vi "Read Configuration File.vi"(8 "error in (no error)":errorcluster, 11 "Instrument.Lockin":refnum<class "Instrument.Lockin.lvclass">) -> (0 "error out":errorcluster, 3 "Instrument.Lockin out":refnum<class "Instrument.Lockin.lvclass">)   [LabVIEW 2019, in "Instrument.Lockin.lvlib" / "Instrument.Lockin.lvclass"]
uses:
  Instrument.Lockin.lvclass
  C:/Program Files (x86)/National Instruments/LabVIEW 2019/user.lib/LevyLab/Instrument Framework/Instrument/Instrument.lvclass
  <userlib>/LevyLab/Instrument Framework/Instrument/Instrument.lvclass/Instrument.ctl
  <userlib>/LevyLab/Configuration/Configuration.lvclass/Configuration.ctl
  Instrument.Lockin.lvclass/Instrument.Lockin.ctl
  <userlib>/LevyLab/Configuration/Write Section.vi
  <userlib>/LevyLab/Instrument Framework/Instrument/Instrument.lvclass
  C:/Program Files (x86)/National Instruments/LabVIEW 2019/vi.lib/JKI/JKI SMO/SMO/SMO.lvclass
  <vilib>/JKI/JKI SMO/SMO/Protected/ThisLevelClassName.vi
  <userlib>/LevyLab/Instrument Framework/Instrument Types/Lockin/Instrument.LockinAPI.lvclass
  <userlib>/LevyLab/Configuration/Configuration.lvclass
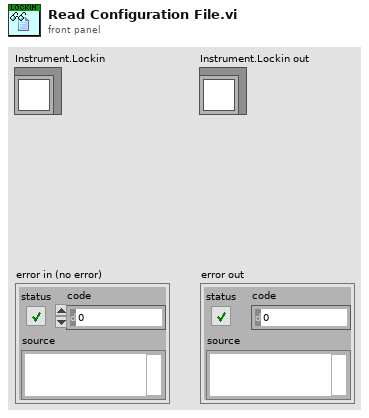
[diagram p1: front panel]
types:
  T1 = typedef "Instrument.Lockin.lvlib/Instrument.Lockin.lvclass/Lockin.Logging Mode--Enum.ctl" = enum16{"enabled", "disabled"}
  T2 = typedef "Instrument.Lockin.lvlib/Instrument.Lockin.lvclass/Lockin.LogPaths.Data--Cluster.ctl" = cluster{"PXI":cluster{"System Serial Number (text)":string, "Channel (i32)":string, "Channel Type (text)":string, "Data (dbl)":string, "Sweeping? (bool)":string}, "MCLI":cluster{"System Serial Number (text)":string, "System Channel (i32)":string, "Ref Channel (i32)":string, "X Data (dbl)":string, "Y Data (dbl)":string, "Sweeping? (bool)":string}}
  T3 = typedef "Instrument.Lockin.lvlib/Instrument.Lockin.lvclass/Lockin.LogPaths.Configuration--Cluster.ctl" = cluster{"Systems":cluster{"System Serial Number (text)":string, "Chassis Serial Number (text)":string, "Chassis Type (text)":string, "Sample Rate (dbl)":string}, "Devices":cluster{"System Serial Number (text)":string, "Chassis Serial Number (text)":string, "Device Serial Number (text)":string, "Device Type (text)":string, "Chassis Slot (i32)":string, "Device Temperature (dbl)":string, "Device Calibration Temperature (dbl)":string, "Device Calibration Time (timestamptz)":string}, "Channels":cluster{"System Serial Number (text)":string, "System Channel (i32)":string, "Device Serial Number (text)":string, "Device Channel (i32)":string, "Channel Type (text)":string, "Channel Coupling (text)":string, "Channel Range (text)":string, "Channel Configuration (text)":string}, "MCLI":cluster{"System Serial Number (text)":string, "Software Version (text)":string, "REF Channel (i32)":string, "frequency (dbl)":string, "time constant (dbl)":string, "roll-off (i32)":string}}
  T4 = cluster{"Loggin mode":T1, "Logging interval (ms)":u32, "Data Log Paths":T2, "Config Log Paths":T3}
  T5 = typedef "Instrument.Lockin.lvlib/Instrument.DAQ.lvclass/Configuration--Cluster.ctl" = cluster{"DAQ":T6, "Channels":T21, "Prefilter":T29, "Offset and Gain":T30, "Amplitude Limit":T33, "DC Limit":T34, "Link Frequencies":T35, "Sweep":T36, "Duty Cycle":T40}
  T6 = typedef "Instrument.Lockin.lvlib/Instrument.DAQ.lvclass/Configuration.DAQ--Cluster.ctl" = cluster{"Sampling":T7, "Simulation mode":T10, "AI":T11, "AO":T16, "Calibration":T18, "Devices":T20[]}
  T7 = typedef "Instrument.Lockin.lvlib/Instrument.DAQ.lvclass/DAQ.Sampling--Cluster.ctl" = cluster{"Sampling":T8, "sample mode":i32, "Fs Mode":T9, "Fs Multiplier":dbl, "Refresh Rate (Hz)":dbl, "Decimation.PreDSP":i32, "Decimation.PostDSP":i32, "Fs.Output":dbl}
  T8 = typedef "Instrument.Lockin.lvlib/Instrument.DAQ.lvclass/DAQ.Sampling.Sampling--Cluster.ctl" = cluster{"Fs":dbl, "#s":i32}
  T9 = typedef "Instrument.Lockin.lvlib/Instrument.DAQ.lvclass/DAQ.Sampling.Fs Mode--enum.ctl" = enum16{"Manual", "Auto Fs", "Max Fs"}
  T10 = typedef "Instrument.Lockin.lvlib/Instrument.DAQ.lvclass/Simulation Mode--enum.ctl" = enum16{"AI = HW simulated", "AI = noise*AO", "AI = waveguide"}
  T11 = typedef "Instrument.Lockin.lvlib/Instrument.DAQ.lvclass/DAQ.Config.AI--Cluster--Array.ctl" = cluster{"Channels":tag, "Coupling":T12, "Range":T13, "terminal configuration":T14, "Type":T15}[]
  T12 = typedef "Instrument.Lockin.lvlib/Instrument.DAQ.lvclass/DAQ.Config.AI.Coupling--enum.ctl" = u16
  T13 = typedef "Instrument.Lockin.lvlib/Instrument.DAQ.lvclass/DAQ.Config.AI.Range--enum.ctl" = enum16{"±0.316", "±1.00", "±3.16", "±10.0", "±31.6", "±42.4", ""}
  T14 = typedef "Instrument.Lockin.lvlib/Instrument.DAQ.lvclass/DAQ.TerminalConfiguration--ring.ctl" = i32
  T15 = typedef "Instrument.Lockin.lvlib/Instrument.DAQ.lvclass/DAQ.Type--enum.ctl" = enum16{"None", "USB-4431", "PXI-446x"}
  T16 = typedef "Instrument.Lockin.lvlib/Instrument.DAQ.lvclass/DAQ.Config.AO--Cluster--Array.ctl" = cluster{"Channels":tag, "Range":T17, "terminal configuration":T14, "Type":T15}[]
  T17 = typedef "Instrument.Lockin.lvlib/Instrument.DAQ.lvclass/DAQ.Config.AO.Range--enum.ctl" = enum16{"±0.1", "±1.0", "±10.0", ""}
  T18 = typedef "Instrument.Lockin.lvlib/Instrument.DAQ.lvclass/DAQ.Calibration--Cluster--Array.ctl" = T19[]
  T19 = typedef "Instrument.Lockin.lvlib/Instrument.DAQ.lvclass/DAQ.Calibration--Cluster.ctl" = cluster{"Active Device":string, "SelfCal.LastDate/Time":dbl, "SelfCal.LastTemp":dbl, "DevTemp":dbl, "calibration due?":bool}
  T20 = typedef "Instrument.Lockin.lvlib/Instrument.DAQ.lvclass/DeviceInfo--Cluster.ctl" = cluster{"DeviceName":string, "DevIsSimulated":bool, "DeviceSerialNumber":string, "ProductType":string, "ProductCategory":i32, "ProductNumber":u32, "ChassisNumber":u32, "SlotNumber":u32, "ChassisName":string, "ChassisSerialNumber":string, "DevTemp":dbl, "SelfCal.LastDate/Time":string, "SelfCal.LastTemp":dbl, "calibration due?":bool}
  T21 = typedef "Instrument.Lockin.lvlib/Instrument.DAQ.lvclass/Configuration.Channels--Cluster.ctl" = cluster{"Cfg_AO":T22, "Cfg_AI":T25, "Cfg_REF":T27}
  T22 = typedef "Instrument.Lockin.lvlib/Instrument.DAQ.lvclass/AO.Channel--Cluster--Array.ctl" = T23[]
  T23 = typedef "Instrument.Lockin.lvlib/Instrument.DAQ.lvclass/AO.Channel--Cluster.ctl" = cluster{"Enable?":bool, "Channel":i32, "Amplitude":dbl, "Offset":dbl, "Frequency":dbl, "Phase":dbl, "Function":T24, "Sweeping?":bool, "Limit AC":bool, "Limit DC?":bool, "Duty Cycle":bool}
  T24 = typedef "Instrument.Lockin.lvlib/Instrument.DAQ.lvclass/AO.Channel.Function--Enum.ctl" = enum16{"sine", "square", "triangle", "saw"}
  T25 = typedef "Instrument.Lockin.lvlib/Instrument.DAQ.lvclass/AI.Channel--Cluster--Array.ctl" = T26[]
  T26 = typedef "Instrument.Lockin.lvlib/Instrument.DAQ.lvclass/AI.Channel--Cluster.ctl" = cluster{"Enable?":bool, "Channel":i32, "References":u16[], "reference index":i32}
  T27 = typedef "Instrument.Lockin.lvlib/Instrument.DAQ.lvclass/REF.Channel--Cluster--Array.ctl" = T28[]
  T28 = typedef "Instrument.Lockin.lvlib/Instrument.DAQ.lvclass/REF.Channel--Cluster.ctl" = cluster{"Enable?":bool, "Channel":i32, "Frequency":dbl, "Phase":dbl, "TC":dbl, "Roll-Off":i32}
  T29 = typedef "Instrument.Lockin.lvlib/Instrument.DAQ.lvclass/Configuration.Prefilter--Cluster.ctl" = cluster{"60 Hz":bool, "Low Pass":bool, "Low Pass Cutoff (Hz)":dbl}
  T30 = typedef "Instrument.Lockin.lvlib/Instrument.DAQ.lvclass/Channel.GainsAndOffsets--Cluster.ctl" = cluster{"Offset_AI":T31, "Gain_AI":T31, "Gain_AO":T31}
  T31 = typedef "Instrument.Lockin.lvlib/Instrument.DAQ.lvclass/Channel.Gain--Cluster--Array.ctl" = T32[]
  T32 = typedef "Instrument.Lockin.lvlib/Instrument.DAQ.lvclass/Channel.Gain--Cluster.ctl" = cluster{"Channel":string, "Gain":dbl}
  T33 = typedef "Instrument.Lockin.lvlib/Instrument.DAQ.lvclass/Configuration.AmplitudeLimit--Cluster.ctl" = cluster{"Limit?":bool, "Limit (V)":dbl}
  T34 = typedef "Instrument.Lockin.lvlib/Instrument.DAQ.lvclass/Configuration.DCLimit--Cluster.ctl" = cluster{"Limit?":bool, "Limit (V)":dbl}
  T35 = typedef "Instrument.Lockin.lvlib/Instrument.DAQ.lvclass/Configuration.LinkFrequencies--Cluster.ctl" = cluster{"Link?":bool, "Frequency (Hz)":dbl}
  T36 = typedef "Instrument.Lockin.lvlib/Instrument.DAQ.lvclass/Sweep.Configuration--Cluster.ctl" = cluster{"Sweep Time (s)":dbl, "Initial Wait (s)":dbl, "Return to Start":bool, "Channels":T37}
  T37 = typedef "Instrument.Lockin.lvlib/Instrument.DAQ.lvclass/Sweep.Channel--Cluster--Array.ctl" = T38[]
  T38 = typedef "Instrument.Lockin.lvlib/Instrument.DAQ.lvclass/Sweep.Channel--Cluster.ctl" = cluster{"Enable?":bool, "Channel":u16, "Start":dbl, "End":dbl, "Pattern":T39, "Table":dbl[]}
  T39 = typedef "Instrument.Lockin.lvlib/Instrument.DAQ.lvclass/Sweep.Pattern--Enum.ctl" = enum16{"Ramp /", "Ramp /\\", "Smooth Ramp _/", "Smooth Ramp _/\\_", "Table"}
  T40 = typedef "Instrument.Lockin.lvlib/Instrument.DAQ.lvclass/Configuration.DutyCycle--Cluster.ctl" = cluster{"Option?":bool, "Duty Cycle (%)":dbl}
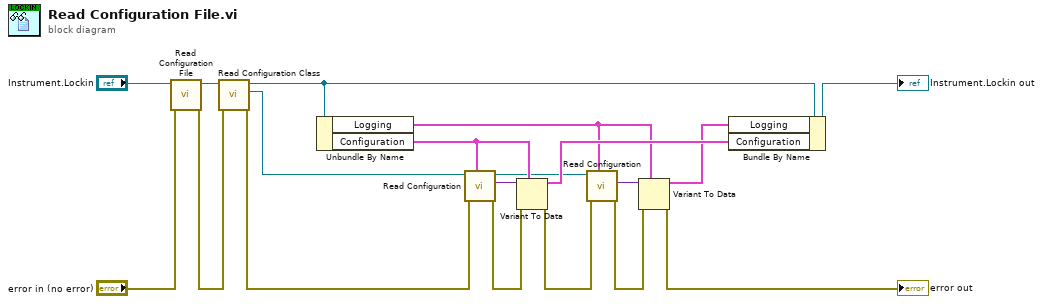
[diagram p0: block diagram]
diagram:
  n1 = call-parent "Read Configuration File.vi"("error in (no error)"="error in (no error)", "Instrument in"="Instrument.Lockin") -> ("error out"=w13:errorcluster, "Instrument out"=w11:refnum<class "Instrument.Lockin.lvclass">)  [unwired: 8 in]
  n2 = call <userlib>:"Read Configuration Class.vi"("error in (no error)"=w13, "Instrument in"=w11) -> ("error out"=w17:errorcluster, "Configuration"=w15:refnum<class "Configuration.lvclass">, "Instrument out"=w3:refnum<class "Instrument.Lockin.lvclass">)  [unwired: 7 in]
  n3 = Unbundle By Name(w3) -> ("Logging"=w6:T4, "Configuration"=w10:T5)
  n4 = call <userlib>:"Read Configuration.vi"("INI Fomatted Cluster Type"=w10, "error in (no error)"=w17, "Configuration in"=w15) -> ("error out"=w18:errorcluster, "Configuration"=w19:variant, "Configuration out"=w9:refnum<class "Configuration.lvclass">)  [unwired: 6 in]
  n5 = Variant To Data(error in=w18, type=w10, Variant=w19) -> (data=w16:T5, error out=w5:errorcluster)
  n6 = call <userlib>:"Read Configuration.vi"("INI Fomatted Cluster Type"=w6, "error in (no error)"=w5, "Configuration in"=w9) -> ("error out"=w4:errorcluster, "Configuration"=w8:variant)  [unwired: 6 in, 1 out]
  n7 = Variant To Data(error in=w4, type=w6, Variant=w8) -> (data=w7:T4, error out=→"error out":errorcluster)
  n8 = Bundle By Name(cluster=w3, "Logging"=w7, "Configuration"=w16) -> (→"Instrument.Lockin out":refnum<class "Instrument.Lockin.lvclass">)
